vi "Drive Used GB.vi"(8 "error in (no error)":errorcluster, 10 "Path":path, 11 "Linux System SAL in":refnum<class "Linux System SAL.lvclass">) -> (0 "error out":errorcluster, 2 "Used GB":dbl, 3 "Linux System SAL out":refnum<class "Linux System SAL.lvclass">)   [LabVIEW 2020, in "Volatus.lvlib" / "Linux System SAL.lvclass"]
uses:
  Linux System SAL.lvclass
  Linux System SAL.lvclass/Linux System SAL.ctl
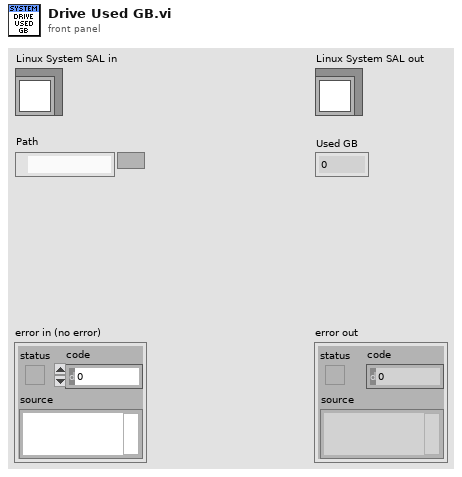
[diagram p1: front panel]
types:
  T1 = typedef "Volatus.lvlib/Linux System SAL.lvclass/Disk Info.ctl" = cluster{"Filesystem":string, "Capacity":dbl, "Used":dbl, "Available":dbl}
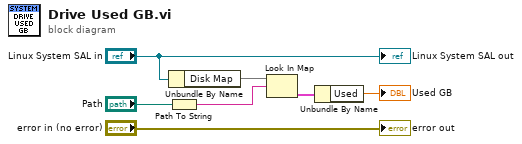
[diagram p0: block diagram]
diagram:
  n1 = Unbundle By Name("Linux System SAL in") -> ("Disk Map"=w4:map{string, T1})
  n2 = Path To String(path="Path") -> (string=w3:string)
  n3 = Look In Map(map=w4, key=w3) -> (value=w2:T1)  [unwired: 1 in, 1 out]
  n4 = Unbundle By Name(w2) -> ("Used"=→"Used GB":dbl)
  "error out" <- "error in (no error)"
  "Linux System SAL out" <- "Linux System SAL in"
